vi "ramp with quintic reset.vi"(8 "Frame Samples":i32=128, 10 "Overshoot Samples":i32=128, 11 "Ramp Samples":i32=128) -> (2 "Scan waveform":dbl[](array[numeric]))   [LabVIEW 2020, in "Scan Generators.lvlib"]
uses:
  <vilib>/Analysis/Matrix/Datatypes/RealMatrix.ctl
  <vilib>/Analysis/1siggen.llb/Ramp Pattern by Samples.vi
  <vilib>/Analysis/7linalg.llb/Solve Linear Equations (single right hand).vi
  <vilib>/Analysis/baseanly.llb/Solve Linear Equations By Cholesky.vi
  <vilib>/Analysis/baseanly.llb/Real Matrix to Compact Array.vi
  <vilib>/Analysis/baseanly.llb/Real Compact Tri-Matrix Linear Eqs.vi
  <vilib>/Analysis/7linalg.llb/Solve Linear Eqs (General).vi
  <vilib>/Analysis/7linalg.llb/Solve Linear Eqs (Gen, single right hand).vi
  <vilib>/Analysis/polynomials.llb/1D Polynomial Evaluation (DBL).vi
  Scan Generators.lvlib
  <vilib>/Analysis/NI_AALBase.lvlib
  <vilib>/Analysis/Matrix/NI_Matrix.lvlib
  <vilib>/Analysis/NI_AALPro.lvlib
panel:
  out "Reset samples":i32
  out "Solution Vector":dbl[](array[numeric]) format="%.2f"
  out "Waveform Graph":dbl[](graph)
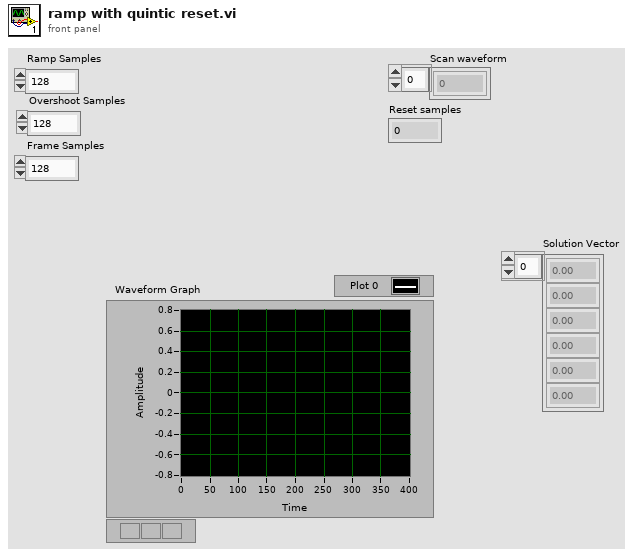
[diagram p1: front panel]
types:
  T1 = typedef "NI_Matrix.lvlib/RealMatrix.ctl" = dbl[][]
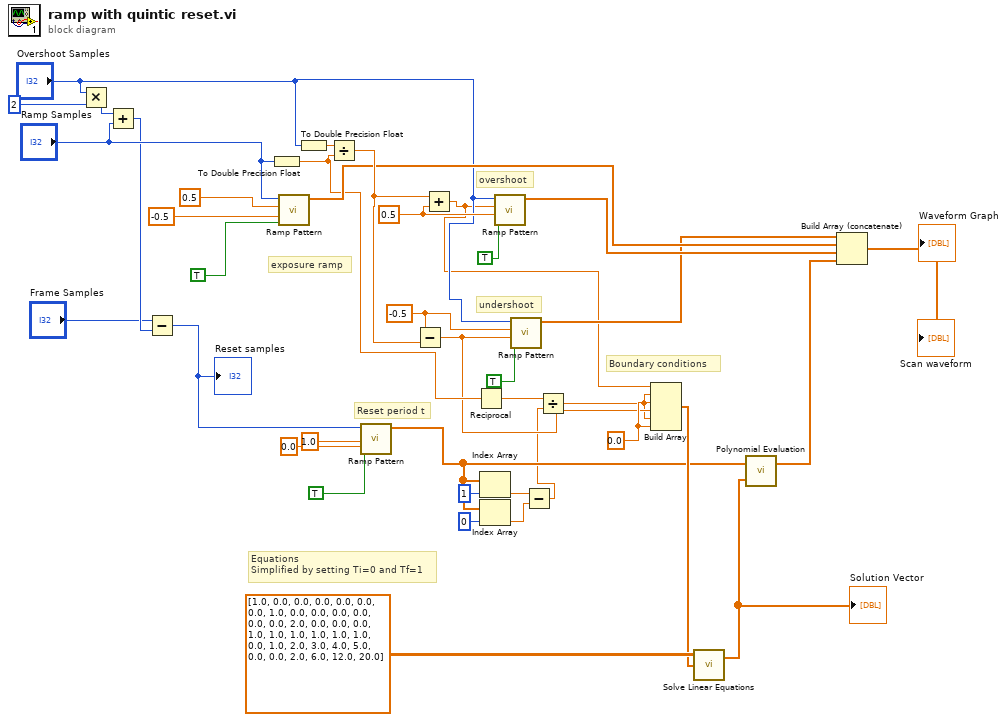
[diagram p0: block diagram]
diagram:
  w15 = 0.0 ("element")
  w33 = -0.5 ("end")
  w32 = 0.5 ("start")
  # "Equations\nSimplified by setting Ti=0 and Tf=1"
  # "Reset period t"
  # "Boundary conditions"
  # "exposure ramp"
  # "undershoot"
  # "overshoot"
  n1 = Multiply(x="Overshoot Samples", y=2) -> (x*y=w24:i32)
  n2 = Add(x=w24, y="Ramp Samples") -> (x+y=w22:i32)
  n3 = Subtract(x="Frame Samples", y=w22) -> (x-y=w17:i32)
  "Reset samples" <- w17
  n4 = To Double Precision Float(number="Ramp Samples") -> (double precision float=w16:dbl)
  n5 = call-poly <vilib>:"Ramp Pattern.vi"("exclude end?"=TRUE, "start"=-0.5, "end"=0.5, "samples"="Ramp Samples") -> ("Ramp Pattern"=w29:dbl[])  [unwired: 6 in, 1 out]
  n6 = To Double Precision Float(number="Overshoot Samples") -> (double precision float=w36:dbl)
  n7 = Divide(x=w36, y=w16) -> (x/y=w30:dbl)
  n8 = call-poly <vilib>:"Ramp Pattern.vi"("exclude end?"=TRUE, "start"=0.0, "end"=1.0, "samples"=w17) -> ("Ramp Pattern"=w8:dbl[])  [unwired: 6 in, 1 out]
  n9 = Subtract(x=w33, y=w30) -> (x-y=w9:dbl)
  n10 = Add(x=w30, y=w32) -> (x+y=w10:dbl)
  n11 = Reciprocal(x=w16) -> (1/x=w3:dbl)
  n12 = Index Array(array=w8, index=1) -> (element=w5:dbl)
  n13 = Index Array(array=w8, index=0) -> (element=w4:dbl)
  n14 = call-poly <vilib>:"Ramp Pattern.vi"("exclude end?"=TRUE, "start"=w32, "end"=w10, "samples"="Overshoot Samples") -> ("Ramp Pattern"=w28:dbl[])  [unwired: 6 in, 1 out]
  n15 = call-poly <vilib>:"Ramp Pattern.vi"("exclude end?"=TRUE, "start"=w9, "end"=w33, "samples"="Overshoot Samples") -> ("Ramp Pattern"=w27:dbl[])  [unwired: 6 in, 1 out]
  n16 = Subtract(x=w5, y=w4) -> (x-y=w2:dbl)
  n17 = Divide(x=w3, y=w2) -> (x/y=w1:dbl)
  n18 = Build Array(w10, w1, w15, w9, w1, w15) -> (w13:dbl[])
  n19 = call-poly <vilib>:"Solve Linear Equations.vi"("Known Vector"=w13, "Input Matrix"=T1 [[1.0, 0.0, 0.0, 0.0, 0.0, 0.0], [0.0, 1.0, 0.0, 0.0, 0.0, 0.0], [0.0, 0.0, 2.0, 0.0, 0.0, 0.0], [1.0, 1.0, 1.0, 1.0, 1.0, 1.0], [0.0, 1.0, 2.0, 3.0, 4.0, 5.0], [0.0, 0.0, 2.0, 6.0, 12.0, 20.0]] ("matrix")) -> ("Solution Vector"=w12:dbl[])  [unwired: 1 in, 1 out]
  "Solution Vector" <- w12
  n20 = call-poly <vilib>:"Polynomial Evaluation.vi"("P(x)"=w12, "A"=w8) -> ("P(A)"=w11:dbl[])  [unwired: 1 out]
  n21 = Build Array (concatenate)(w27, w29, w28, w11) -> (→"Waveform Graph" →"Scan waveform":dbl[])
